vi "ALL - CE-Math VIs.vi"   [LabVIEW 2021]
doc: "::: CalcExpress Toolkit :::\nCopyright (c) 2000-2026 Konstantin Shifershteyn. All rights reserved."
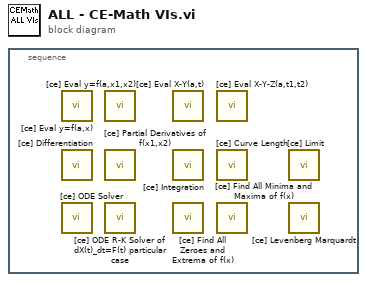
[diagram p0: block diagram]
diagram:
  n1 = stacked-sequence {
    frame #0 {
      n2 = call "[ce] Eval y=f(a,x).vi"() -> ()  [unwired: 8 in, 4 out]
      n3 = call "[ce] Differentiation.vi"() -> ()  [unwired: 7 in, 5 out]
      n4 = call "[ce] ODE Solver.vi"() -> ()  [unwired: 8 in, 4 out]
      n5 = call "[ce] Eval y=f(a,x1,x2).vi"() -> ()  [unwired: 7 in, 5 out]
      n6 = call "[ce] Partial Derivatives of f(x1,x2).vi"() -> ()  [unwired: 7 in, 5 out]
      n7 = call "[ce] ODE R-K Solver of dX(t)_dt=F(t) particular case.vi"() -> ()  [unwired: 8 in, 4 out]
      n8 = call "[ce] Eval X-Y(a,t).vi"() -> ()  [unwired: 8 in, 4 out]
      n9 = call "[ce] Integration.vi"() -> ()  [unwired: 7 in, 5 out]
      n10 = call "[ce] Find All Zeroes and Extrema of f(x).vi"() -> ()  [unwired: 7 in, 5 out]
      n11 = call "[ce] Eval X-Y-Z(a,t1,t2).vi"() -> ()  [unwired: 7 in, 5 out]
      n12 = call "[ce] Curve Length.vi"() -> ()  [unwired: 8 in, 4 out]
      n13 = call "[ce] Find All Minima and Maxima of f(x).vi"() -> ()  [unwired: 8 in, 4 out]
      n14 = call "[ce] Limit.vi"() -> ()  [unwired: 6 in, 4 out]
      n15 = call "[ce] Levenberg Marquardt.vi"() -> ()  [unwired: 9 in, 7 out]
    }
  }
